vi "insert_node.vi"(9 "node":refnum<class "Node.lvclass">, 11 "graph":refnum<class "Graph.lvclass">) -> (1 "node unchanged?":bool, 2 "node already included?":bool, 3 "graph out":refnum<class "Graph.lvclass">)   [LabVIEW 2020, in "graph.lvlib" / "Graph.lvclass"]
uses:
  Graph.lvclass
  Node/Node.lvclass
  Node/Node.lvclass/Node.ctl
  Graph.lvclass/Graph.ctl
  lookup_node_index_by_id.vi
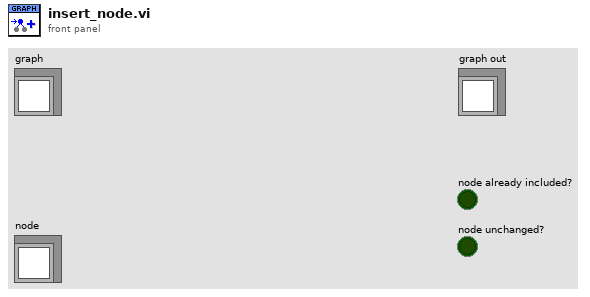
[diagram p1: front panel]
types:
  T1 = map{refnum<class "ID.lvclass">, refnum<class "Node.lvclass">}
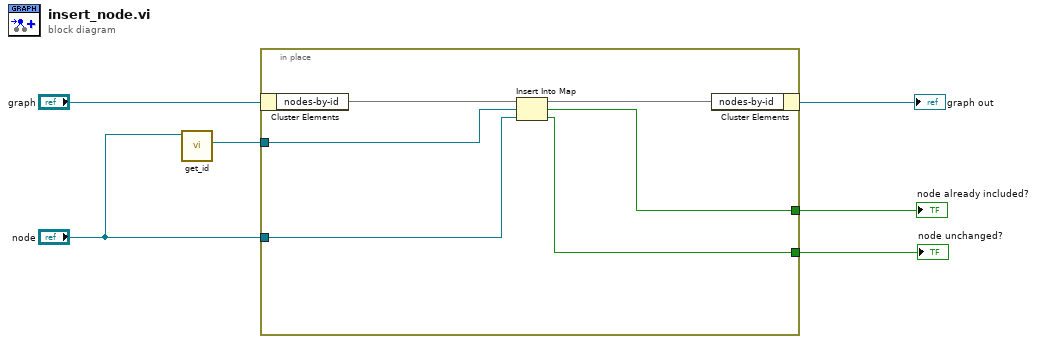
[diagram p0: block diagram]
diagram:
  n1 = call "get_id.vi"("node"="node") -> ("node-id"=w1:refnum<class "ID.lvclass">)  [unwired: 10 in]
  n2 = in-place {
    in-place-border: "node" -> [w11]
    in-place-border: [w9] -> w5
    in-place-border: [w8] -> w4
    in-place-border: w1 -> [w7]
    n3 = in-place-cluster #1("graph") -> ("nodes-by-id"=w12:T1)
    n4 = Insert Into Map(map in=w12, key=w7, value=w11) -> (map out=w10:T1, key already included?=w8:bool, value unchanged?=w9:bool)
    n5 = in-place-cluster #1("nodes-by-id"=w10) -> (→"graph out":refnum<class "Graph.lvclass">)
  }
  "node unchanged?" <- w5
  "node already included?" <- w4
